vi "Report Earnings.vi"(11 "market":T1) -> (3 "market out":T1)   [LabVIEW 2020, in "Full Featured MCP Server.lvlib"]
doc: "Every 60 seconds one company reports its quarterly numbers, one after the other. The surprise is random and leans with the quality of the company; the bigger the surprise, the bigger the move."
uses:
  Full Featured MCP Server.lvlib
  Market State.ctl
  News Item.ctl
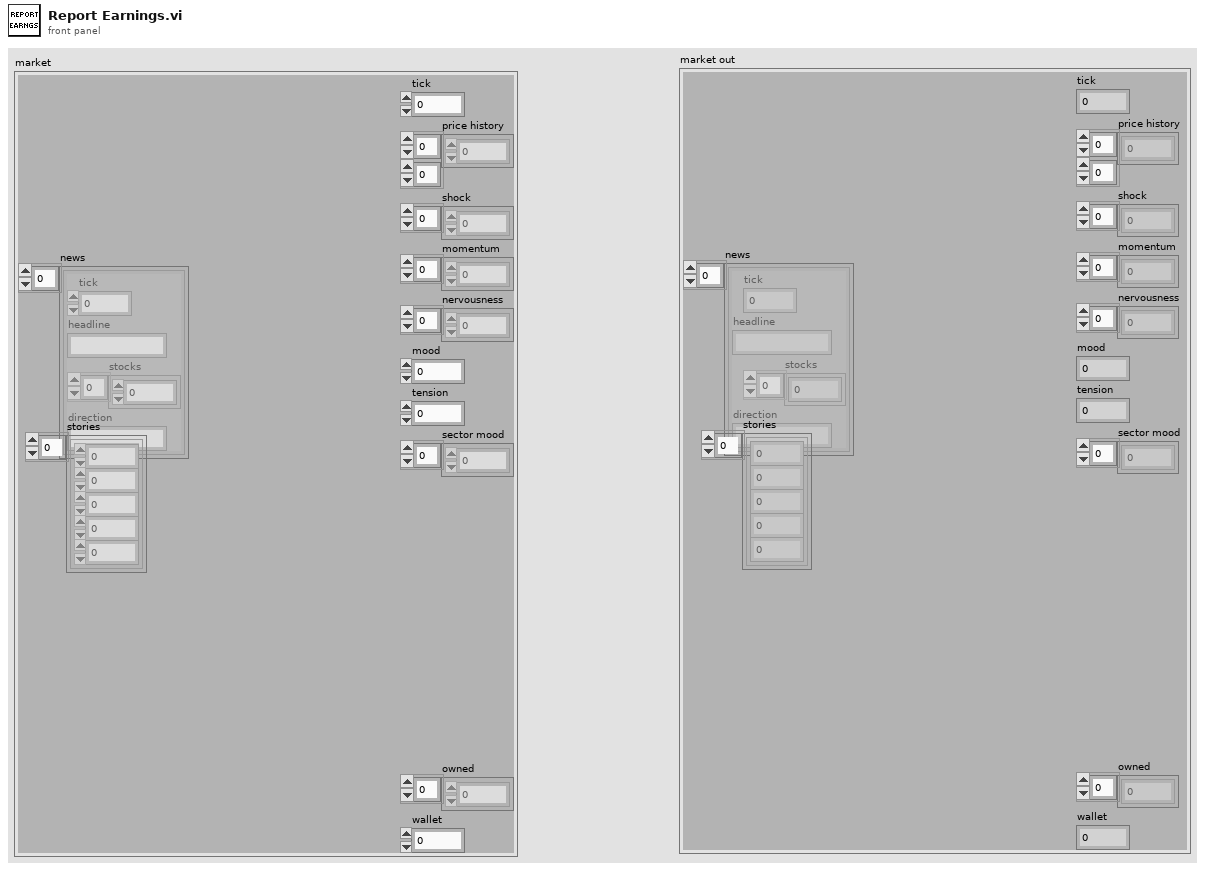
[diagram p1: front panel]
types:
  T1 = typedef "Full Featured MCP Server.lvlib/Market State.ctl" = cluster{"tick":i32, "price history":dbl[][], "shock":dbl[], "momentum":dbl[], "nervousness":dbl[], "mood":dbl, "tension":dbl, "sector mood":dbl[], "news":T2[], "stories":cluster{"arc":i32, "step":i32, "due":i32, "stock":i32, "other":i32}[], "owned":i32[], "wallet":dbl}
  T2 = typedef "Full Featured MCP Server.lvlib/News Item.ctl" = cluster{"tick":i32, "headline":string, "stocks":i32[], "direction":string}
  T3 = cluster{"name":string, "sector":i32, "quality":i32, "start price":dbl, "drift":dbl, "volatility":dbl, "beta":dbl, "jumpiness":dbl, "description":string}[]
  T4 = cluster{"headline":string, "scope":enum16{"one stock", "two stocks", "sector", "market"}, "direction":string, "jump":dbl, "follow":dbl, "jump other":dbl, "follow other":dbl}[]
  T5 = cluster{"name":string, "sector":i32, "quality":i32, "start price":dbl, "drift":dbl, "volatility":dbl, "beta":dbl, "jumpiness":dbl, "description":string}
  T6 = cluster{"headline":string, "scope":enum16{"one stock", "two stocks", "sector", "market"}, "direction":string, "jump":dbl, "follow":dbl, "jump other":dbl, "follow other":dbl}
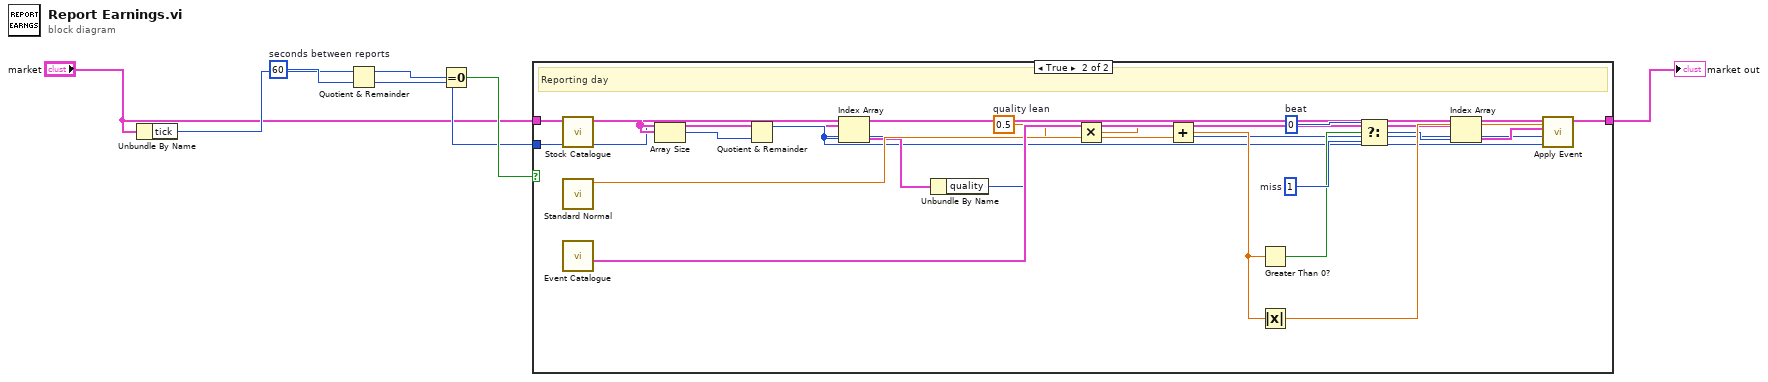
[diagram p0: block diagram]
diagram:
  w3 = 60  # seconds between reports
  n1 = Unbundle By Name("market") -> ("tick"=w2:i32)
  n2 = Quotient & Remainder(x=w2, y=w3) -> (x-y*floor(x/y)=w4:i32, floor(x/y)=w5:i32)
  n3 = Equal To 0?(x=w4) -> (x = 0?=w6:bool)
  n4 = case shown="True" w6 {
    tunnel: "market" -> [w8 w10]
    tunnel: w5 -> [_ w9]
    tunnel: [w8 w11] -> w7
    frame False {
      # "No report"
    }
    frame True {
      w24 = 1  # miss
      w23 = 0  # beat
      w17 = 0.5  # quality lean
      # "Reporting day"
      n5 = call "Stock Catalogue.vi"() -> ("stocks"=w12:T3)  [unwired: 10 in, 1 out]
      n6 = call "Standard Normal.vi"() -> ("number"=w19:dbl)  [unwired: 11 in]
      n7 = call "Event Catalogue.vi"() -> ("earnings"=w21:T4)  [unwired: 8 in, 3 out]
      n8 = Array Size(array=w12) -> (size(s)=w13:i32)
      n9 = Quotient & Remainder(x=w9, y=w13) -> (x-y*floor(x/y)=w14:i32)  [unwired: 1 out]
      n10 = Index Array(array=w12, index=w14) -> (element=w15:T5)
      n11 = Unbundle By Name(w15) -> ("quality"=w16:i32)
      n12 = Multiply(x=w16, y=w17) -> (x*y=w18:dbl)
      n13 = Add(x=w18, y=w19) -> (x+y=w20:dbl)
      n14 = Greater Than 0?(x=w20) -> (x > 0?=w22:bool)
      n15 = Absolute Value(x=w20) -> (abs(x)=w27:dbl)
      n16 = Select(t=w23, s=w22, f=w24) -> (s? t:f=w25:i32)
      n17 = Index Array(array=w21, index=w25) -> (element=w26:T6)
      n18 = call "Apply Event.vi"("scale"=w27, "other"=w14, "stock"=w14, "event"=w26, "market"=w10) -> ("market out"=w11:T1)  [unwired: 6 in]
    }
  }
  "market out" <- w7
